vi "Arreglo_Bidimensional_Subarreglo.vi"() -> ()   [LabVIEW 2026]
panel:
  in  "VALORES NUEVOS":dbl[](array[numeric])
  out "INDICADOR":dbl[][](array[numeric])
  in  "COLUMNA":i16
  in  "ORIGINAL":dbl[][](array[numeric])
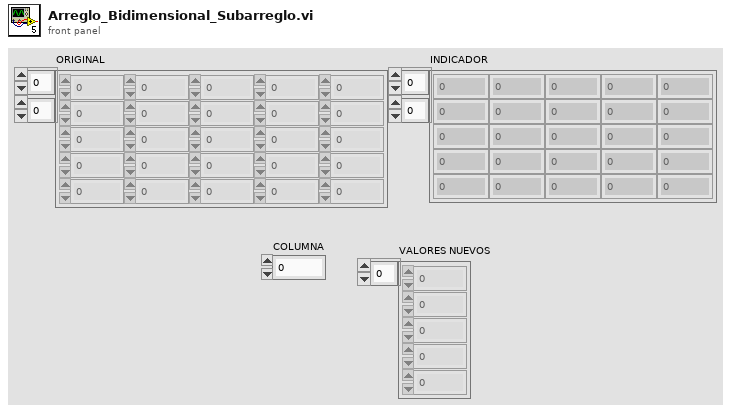
[diagram p1: front panel]
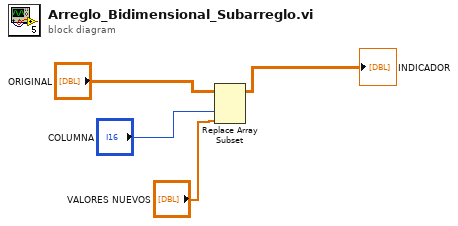
[diagram p0: block diagram]
diagram:
  n1 = Replace Array Subset(array="ORIGINAL", new element="VALORES NUEVOS", index (col)="COLUMNA") -> (→"INDICADOR":dbl[][])  [unwired: 1 in]
